vi "Audio_Start.vi"(11 "error in":errorcluster) -> (4 "Bank":cluster{"Y":dbl[]}[](array[cluster]), 6 "Task ID":u32, 8 "Mixer":T1={"Current"=[], "Position"=0, "Priority"=99, "Music"=FALSE, "MusicPos"=0}, 15 "error out":errorcluster)   [LabVIEW 2020, in "GH_App.lvlib"]
doc: "Loads all sounds (Sound_Bank_Load) and opens a continuous sound channel (22050 Hz, mono, 16 bit, buffer 2048 samples). Also returns the empty mixer state."
uses:
  GH_App.lvlib
  Audio/GH_Audio.lvlib
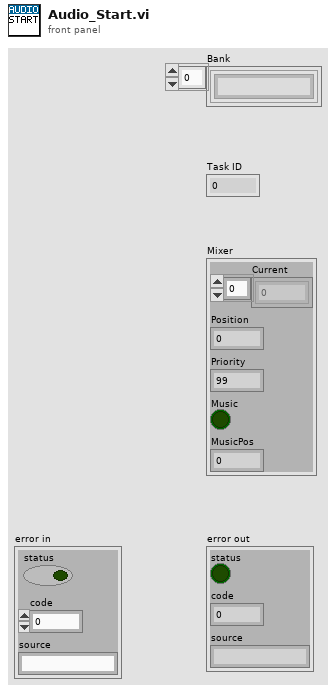
[diagram p1: front panel]
types:
  T1 = cluster{"Current":dbl[], "Position":i32, "Priority":i32, "Music":bool, "MusicPos":i32}
  T2 = cluster{"sample rate (S/s)":dbl, "number of channels":i32, "bits per sample":i32}
  T3 = typedef "Sound Output Task ID.ctl" = u32
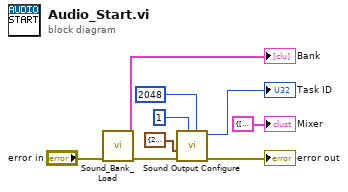
[diagram p0: block diagram]
diagram:
  n1 = call "Sound_Bank_Load.vi"("error in"="error in") -> ("Bank"=→"Bank":cluster{"Y":dbl[]}[], "error out"=w3:errorcluster)  [unwired: 13 in]
  n2 = call <vilib>:"Sound Output Configure.vi"("number of samples/ch"=2048 ("Buffer"), "sample mode"=1 ("continuous"), "error in (no error)"=w3, "sound format"=T2 {"sample rate (S/s)"=22050.0, "number of channels"=1, "bits per sample"=16} ("Sound format")) -> ("error out"=→"error out":errorcluster, "task ID"=→"Task ID":T3)  [unwired: 6 in]
  "Mixer" <- T1 {"Current"=[], "Position"=0, "Priority"=99, "Music"=FALSE, "MusicPos"=0} ("Empty mixer")
